vi "Set Display Format and Precision Method.vi"(0 "Display State In":T1={"Measure ?"=[], "Direction"=[], "Loop ?"={"Start"=0, "Finish"=2}, "Storage Location"=[], "Show Current Location"=FALSE, "Current Location"=0, "Show y=0"=FALSE, "Program"=[], "Index"=0, "Average During Loop ?"=FALSE, "# of Loops"=1, "Loop Control"={0, 2}, "Units"="", "Digits"=0, "Significant Figures (F) or DP (T)"=FALSE, "Rate Mode"=FALSE, "Current Y value"=0.0, "Initial Value"=0.0, "Rate Unit"=""} {"# of Loops" min=1 step=1; "Index" min=0 step=1; "Program"."Step" min=0.001 max=80.0 step=0.001 format="%.2f"; "Program"."Target" format="%.2f"}, 1 "Units":string, 5 "Precision":i32=3, 7 "s.f. (F) or d.p.(T)":bool, 9 "Container State":T2, 11 "error in (no error)":errorcluster, 12 "Rate unit":string) -> (4 "Display State Out":T1={"Measure ?"=[], "Direction"=[], "Loop ?"={"Start"=0, "Finish"=2}, "Storage Location"=[], "Show Current Location"=FALSE, "Current Location"=0, "Show y=0"=FALSE, "Program"=[], "Index"=0, "Average During Loop ?"=FALSE, "# of Loops"=1, "Loop Control"={0, 2}, "Units"="", "Digits"=0, "Significant Figures (F) or DP (T)"=FALSE, "Rate Mode"=FALSE, "Current Y value"=0.0, "Initial Value"=0.0, "Rate Unit"=""} {"# of Loops" min=1 step=1; "Index" min=0 step=1; "Program"."Step" min=0.001 max=80.0 step=0.001 format="%.2f"; "Program"."Target" format="%.2f"}, 15 "error out":errorcluster)   [LabVIEW 2012, in "Multi Segment Waveform.xctl"]
uses:
  Multi Segment Waveform.xctl
  <vilib>/_xctls/Container State.ctl
  State.ctl
  <vilib>/_xctls/XControlSupport.lvlib
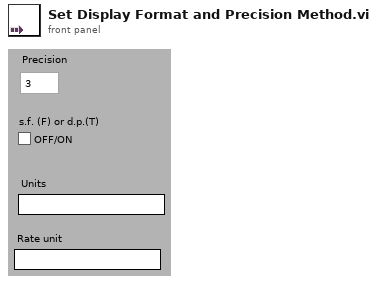
[diagram p1: front panel]
types:
  T1 = typedef "Multi Segment Waveform.xctl/State.ctl" = cluster{"Measure ?":bool[], "Direction":bool[], "Loop ?":cluster{"Start":i32, "Finish":i32}, "Storage Location":i32[], "Show Current Location":bool, "Current Location":i32, "Show y=0":bool, "Program":cluster{"Target":dbl, "Step":dbl, "Measure ?":bool}[], "Index":i32, "Average During Loop ?":bool, "# of Loops":u32, "Loop Control":cluster{i32, i32}, "Units":string, "Digits":i32, "Significant Figures (F) or DP (T)":bool, "Rate Mode":bool, "Current Y value":dbl, "Initial Value":dbl, "Rate Unit":string}
  T2 = typedef "XControlSupport.lvlib/Container State.ctl" = cluster{"Indicator?":bool, "Run Mode?":bool, " Refnum":refnum<vi>}
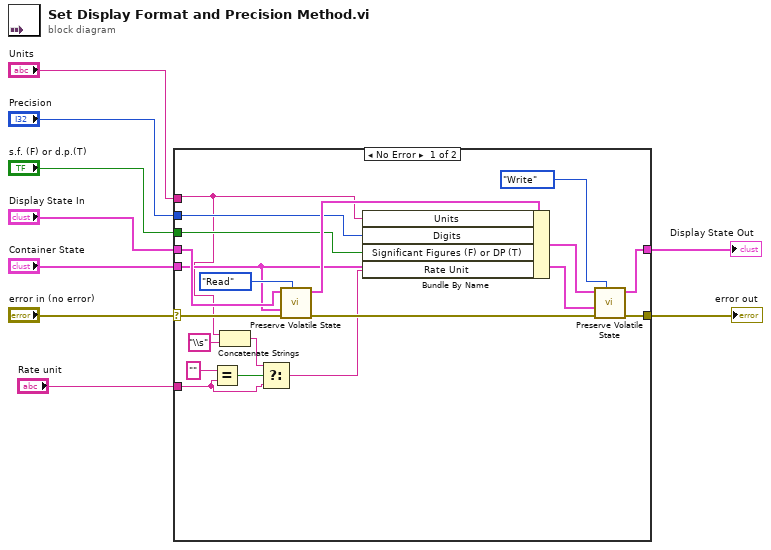
[diagram p0: block diagram]
diagram:
  n1 = case shown="No Error" "error in (no error)" {
    selector: "error in (no error)" -> [w26 w30]
    tunnel: "Display State In" -> [w28 w29]
    tunnel: "Container State" -> [w21 _]
    tunnel: "Units" -> [w13 _]
    tunnel: "Precision" -> [w24 _]
    tunnel: "s.f. (F) or d.p.(T)" -> [w23 _]
    tunnel: [w18 w30] -> w3
    tunnel: [w17 w29] -> w2
    tunnel: "Rate unit" -> [w14 _]
    frame No Error {
      n2 = Equal?(x="", y=w14) -> (x = y?=w15:bool)
      n3 = Concatenate Strings(w13, "\\s" ("string")) -> (w11:string)
      n4 = Select(t=w11, s=w15, f=w14) -> (s? t:f=w10:string)
      n5 = call "Preserve Volatile State.vi"("Operation"=enum16{"Read", "Write", "Update From Data"}."Read", "error in (no error)"=w26, "Container State"=w21, "Waveform State In"=w28) -> ("error out"=w20:errorcluster, "Waveform State Out"=w25:T1)  [unwired: 1 in, 5 out]
      n6 = Bundle By Name(cluster=w25, "Units"=w13, "Digits"=w24, "Significant Figures (F) or DP (T)"=w23, "Rate Unit"=w10) -> (w22:T1)
      n7 = call "Preserve Volatile State.vi"("Operation"=enum16{"Read", "Write", "Update From Data"}."Write", "error in (no error)"=w20, "Container State"=w21, "Waveform State In"=w22) -> ("error out"=w18:errorcluster, "Waveform State Out"=w17:T1)  [unwired: 1 in, 5 out]
    }
    frame Error {
    }
  }
  "Display State Out" <- w2
  "error out" <- w3
